vi "VIH Project - Menu - Build Examples Menu.vi"(8 "error in":errorcluster, 10 "Examples folder":path, 11 "menu reference":refnum<k9>) -> (0 "error out":errorcluster, 3 "dup menu reference":refnum<k9>)   [LabVIEW 2014]
doc: "::: VI Helpeks :::\nCopyright (c) 2000-2026 Konstantin Shifershteyn. All rights reserved."
panel:
  # "VI Helpeks\nCopyright (c) 2012-2026 Konstantin Shifershteyn"
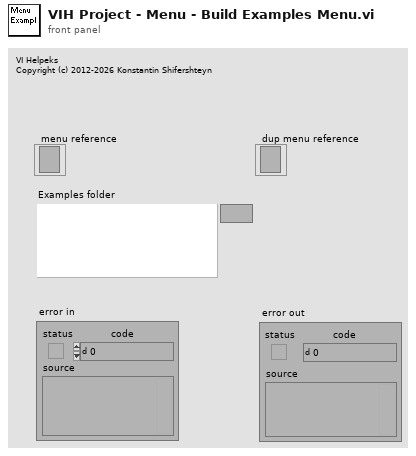
[diagram p1: front panel]
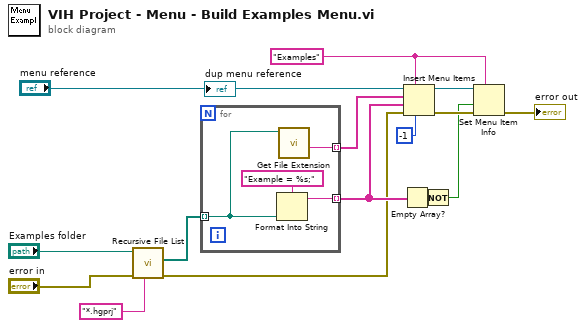
[diagram p0: block diagram]
diagram:
  w8 = "Examples"
  n1 = call <vilib>:"Recursive File List.vi"("pattern"="*.hgprj", "error in (no error)"="error in", "Folder Path"="Examples folder") -> ("error out"=w4:errorcluster, "All Files in Dir"=w12:path[])  [unwired: 4 in, 3 out]
  n2 = for {
    tunnel: w12 -> [w17] mode=indexing
    tunnel: [w18] -> w7 mode=indexing
    tunnel: [w16] -> w11 mode=indexing
    n3 = Format Into String(format string="Example = %s;", w17) -> (resulting string=w18:string)  [unwired: 2 in, 1 out]
    n4 = call <vilib>:"Get File Extension.vi"("file"=w17) -> ("filename without extension"=w16:string)  [unwired: 7 in, 3 out]
  }
  n5 = Empty Array?(array=w7) -> (empty?=w6:bool)
  n6 = Insert Menu Items(4:-1, 5:w8, 6:w4, 7:w7, 8:w11, 9:"menu reference") -> (0:w9:errorcluster, 3:w10:refnum<k9>)  [unwired: 1 out]
  n7 = Not(x=w6) -> (.not. x?=w1:bool)
  n8 = Set Menu Item Info(7:w8, 8:w9, 9:w1, 11:w10) -> (0:→"error out":errorcluster)  [unwired: 3 in, 1 out]
